vi "VIH Project Tree - Defer Panel Updates.vi"(8 "error in":errorcluster, 10 "Defer Panel Updates (F)":bool, 11 "Project Tree":T1) -> (0 "error out":errorcluster, 2 "Previous Defer status":bool, 3 "dup Project Tree":T1)   [LabVIEW 2014]
doc: "::: VI Helpeks :::\nCopyright (c) 2000-2026 Konstantin Shifershteyn. All rights reserved."
uses:
  VIH Project Tree Typedef - Tree Refnum.ctl
panel:
  # "VI Helpeks\nCopyright (c) 2012-2026 Konstantin Shifershteyn"
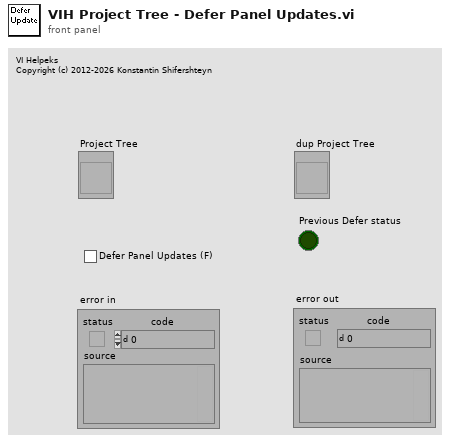
[diagram p1: front panel]
types:
  T1 = typedef "VIH Project Tree Typedef - Tree Refnum.ctl" = refnum<vi>
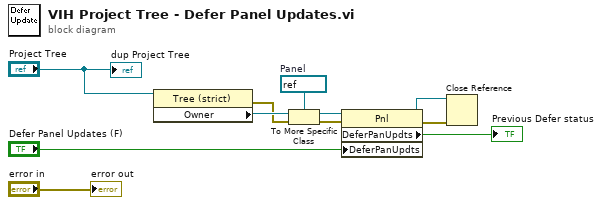
[diagram p0: block diagram]
diagram:
  w10 = refnum<vi> refnum  # Panel
  n1 = property class="Tree (strict)"(reference="Project Tree") -> (error out=w7:errorcluster, "Owner"=w9:refnum<vi>)  [unwired: 1 in, 1 out]
  n2 = To More Specific Class(target class=w10, reference=w9, error in=w7) -> (specific class reference=w11:refnum<vi>, error out=w6:errorcluster)
  n3 = property class="Pnl"(reference=w11, error in=w6, "DeferPanUpdts"="Defer Panel Updates (F)") -> (reference out=w4:refnum<vi>, error out=w3:errorcluster, "DeferPanUpdts"=→"Previous Defer status":bool)
  n4 = Close Reference(reference=w4, error in (no error)=w3) -> ()  [unwired: 1 out]
  "dup Project Tree" <- "Project Tree"
  "error out" <- "error in"
